vi "GetITool.vi"() -> (3 "ITool.lvclass out":refnum<class "ITool.lvclass">)   [LabVIEW 2017]
uses:
  ITool/ITool.lvclass
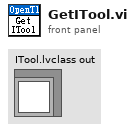
[diagram p1: front panel]
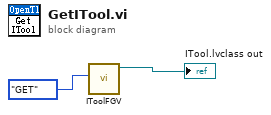
[diagram p0: block diagram]
diagram:
  n1 = call "IToolFGV.vi"("Action"=enum16{"GET", "SET"}."GET") -> ("ITool.lvclass out"=→"ITool.lvclass out":refnum<class "ITool.lvclass">)  [unwired: 10 in]
